vi "Generate Filename.vi"(8 "error in":errorcluster, 10 "Folder":path, 11 "Virtual Instrument in":refnum<class "Virtual Instrument.lvclass">) -> (0 "error out":errorcluster, 2 "File Path":path, 3 "Virtual Instrument out":refnum<class "Virtual Instrument.lvclass">)   [LabVIEW 2026, in "Virtual Instrument.lvclass"]
doc: "This VI generates a file path suitable for saving files based on the provided folder and the implementing classes properties."
uses:
  Virtual Instrument.lvclass
  LabVIEW File/LabVIEW File.lvclass/LabVIEW File.ctl
  LabVIEW File/Read Name.vi
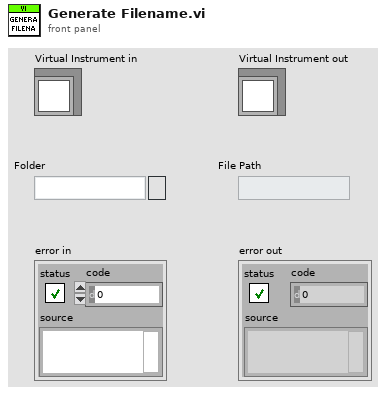
[diagram p1: front panel]
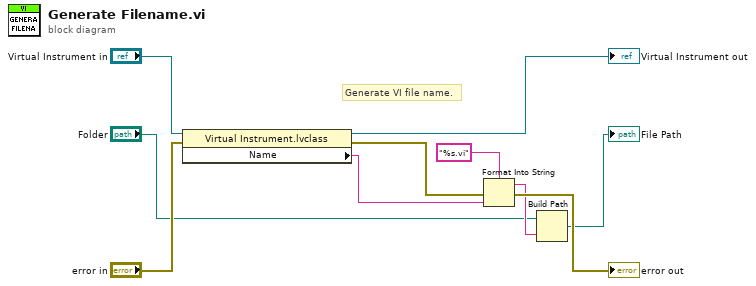
[diagram p0: block diagram]
diagram:
  # "Generate VI file name."
  n1 = property class="Virtual Instrument.lvclass"(reference="Virtual Instrument in", error in="error in") -> (reference out=→"Virtual Instrument out":refnum<class "Virtual Instrument.lvclass">, error out=w9:errorcluster, "Name"=w1:string)
  n2 = Format Into String(format string="%s.vi", error in=w9, w1) -> (resulting string=w6:string, error out=→"error out":errorcluster)  [unwired: 1 in]
  n3 = Build Path(base path="Folder", name or relative path=w6) -> (appended path=→"File Path":path)
